vi "PLC_ReadWords.vi"(8 "error in (no error)":errorcluster, 9 "Count":u16, 10 "Start D":u16, 11 "PLC Conn":refnum<visa-resource-name>) -> (0 "error out":errorcluster, 2 "Words":u16[](array[numeric]), 3 "PLC Conn out":refnum<visa-resource-name>)   [LabVIEW 2018]
doc: "Use this template to build a VI to use as a subVI."
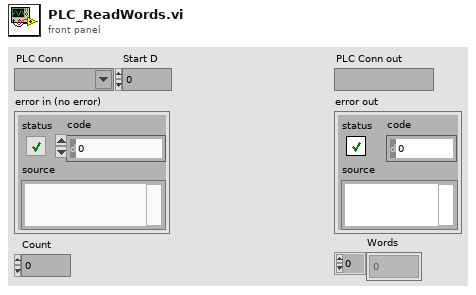
[diagram p1: front panel]
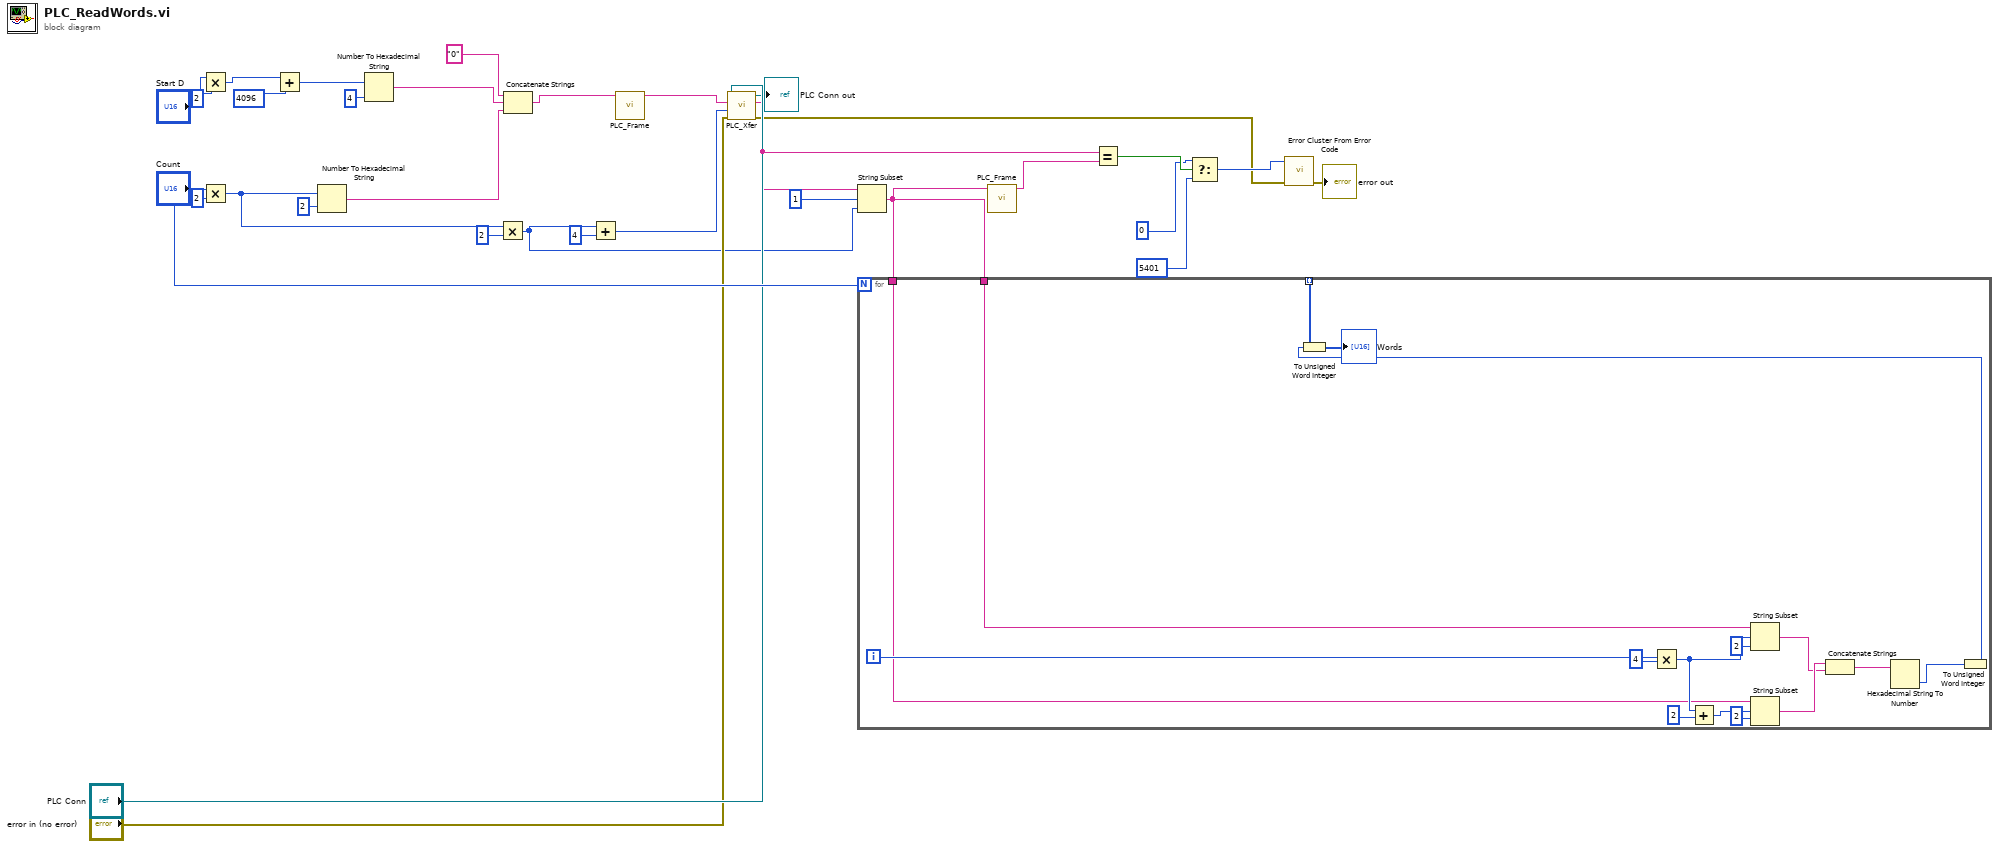
[diagram p0: block diagram]
diagram:
  n1 = Multiply(x="Start D", y=u16 2) -> (x*y=w30:u16)
  n2 = Multiply(x="Count", y=u16 2) -> (x*y=w26:u16)
  n3 = Add(x=w30, y=u16 4096) -> (x+y=w28:u16)
  n4 = Number To Hexadecimal String(1:i16 2 ("width (-)"), 2:w26) -> (0:w22:string)
  n5 = Number To Hexadecimal String(1:i16 4 ("width (-)"), 2:w28) -> (0:w23:string)
  n6 = Multiply(x=w26, y=u16 2) -> (x*y=w16:u16)
  n7 = Concatenate Strings("0", w23, w22) -> (w21:string)
  n8 = Add(x=w16, y=u16 4) -> (x+y=w14:u16)
  n9 = call "PLC_Frame.vi"("Payload"=w21) -> ("Frame"=w20:string)  [unwired: 10 in]
  n10 = call "PLC_Xfer.vi"("error in (no error)"="error in (no error)", "RX Bytes"=w14, "TX"=w20, "PLC Conn"="PLC Conn") -> ("error out"=w6:errorcluster, "RX"=w13:string, "PLC Conn out"=→"PLC Conn out":refnum<visa-resource-name>)  [unwired: 5 in]
  n11 = String Subset(string=w13, offset (0)=1, length (rest)=w16) -> (substring=w3:string)
  n12 = for {
    N: "Count" -> [_]
    tunnel: w3 -> [w46]
    tunnel: w3 -> [w42]
    tunnel: [w35] -> w2 mode=indexing
    i -> [w48]
    n13 = Multiply(x=w48, y=4) -> (x*y=w45:i32)
    n14 = Add(x=w45, y=2) -> (x+y=w41:i32)
    n15 = String Subset(string=w46, offset (0)=w45, length (rest)=2 ("length (rest)")) -> (substring=w38:string)
    n16 = String Subset(string=w42, offset (0)=w41, length (rest)=2 ("length (rest)")) -> (substring=w39:string)
    n17 = Concatenate Strings(w39, w38) -> (w37:string)
    n18 = Hexadecimal String To Number(string=w37) -> (number=w36:u32)  [unwired: 2 in, 1 out]
    n19 = To Unsigned Word Integer(number=w36) -> (unsigned 16bit integer=w35:u16)
  }
  n20 = call "PLC_Frame.vi"("Payload"=w3) -> ("Frame"=w11:string)  [unwired: 10 in]
  n21 = Equal?(x=w13, y=w11) -> (x = y?=w10:bool)
  n22 = Select(t=0, s=w10, f=5401) -> (s? t:f=w7:i32)
  n23 = call <vilib>:"Error Cluster From Error Code.vi"("error in (no error)"=w6, "error code (0)"=w7) -> ("error out"=→"error out":errorcluster)  [unwired: 7 in]
  n24 = To Unsigned Word Integer(number=w2) -> (unsigned 16bit integer=→"Words":u16[])
